vi "SC Save Modified VIs.vi"(8 "error in (no error)":errorcluster, 9 "project folder":path, 10 "project application":refnum<vi>) -> (0 "error out":errorcluster, 1 "cancelled?":bool)   [LabVIEW 2023]
doc: "Before a deploy: lists the VIs in the project's application instance (project application, from SC Get Project) that are inside the project folder and have unsaved changes, and the untitled (never saved) VIs there, asks Save All / Cancel, then asks where to save each untitled VI (starting in the project folder) and saves them all. Untitled VIs are saved first, because saving a caller of an untitled subVI fails. Cancelling any of it cancels the deploy. Unless cancelled, also saves the active project (LabVIEW has no public 'project modified' property)."
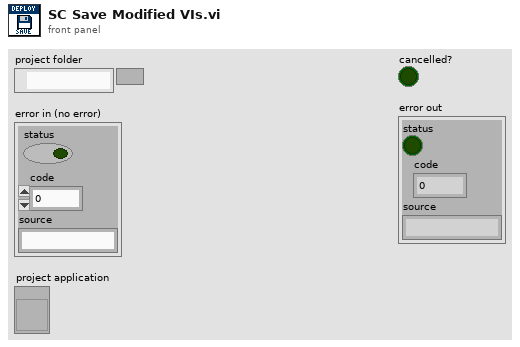
[diagram p1: front panel]
types:
  T1 = enum32{"existing file", "new file", "new or existing file", "existing dir", "new dir", "new or existing dir", "existing file (use LLBs)", "new file (use LLBs)", "new or existing file (use LLBs)", "new or existing file or directory (use LLBs)", "existing dir (use LLBs)", "new dir (use LLBs)", "new or existing dir (use LLBs)", "existing file or dir", "new file or dir", "new or existing file or dir", "existing file or dir (use LLBs)", "new file or dir (use LLBs)", "multi-select", "multi-select (use LLBs)"}
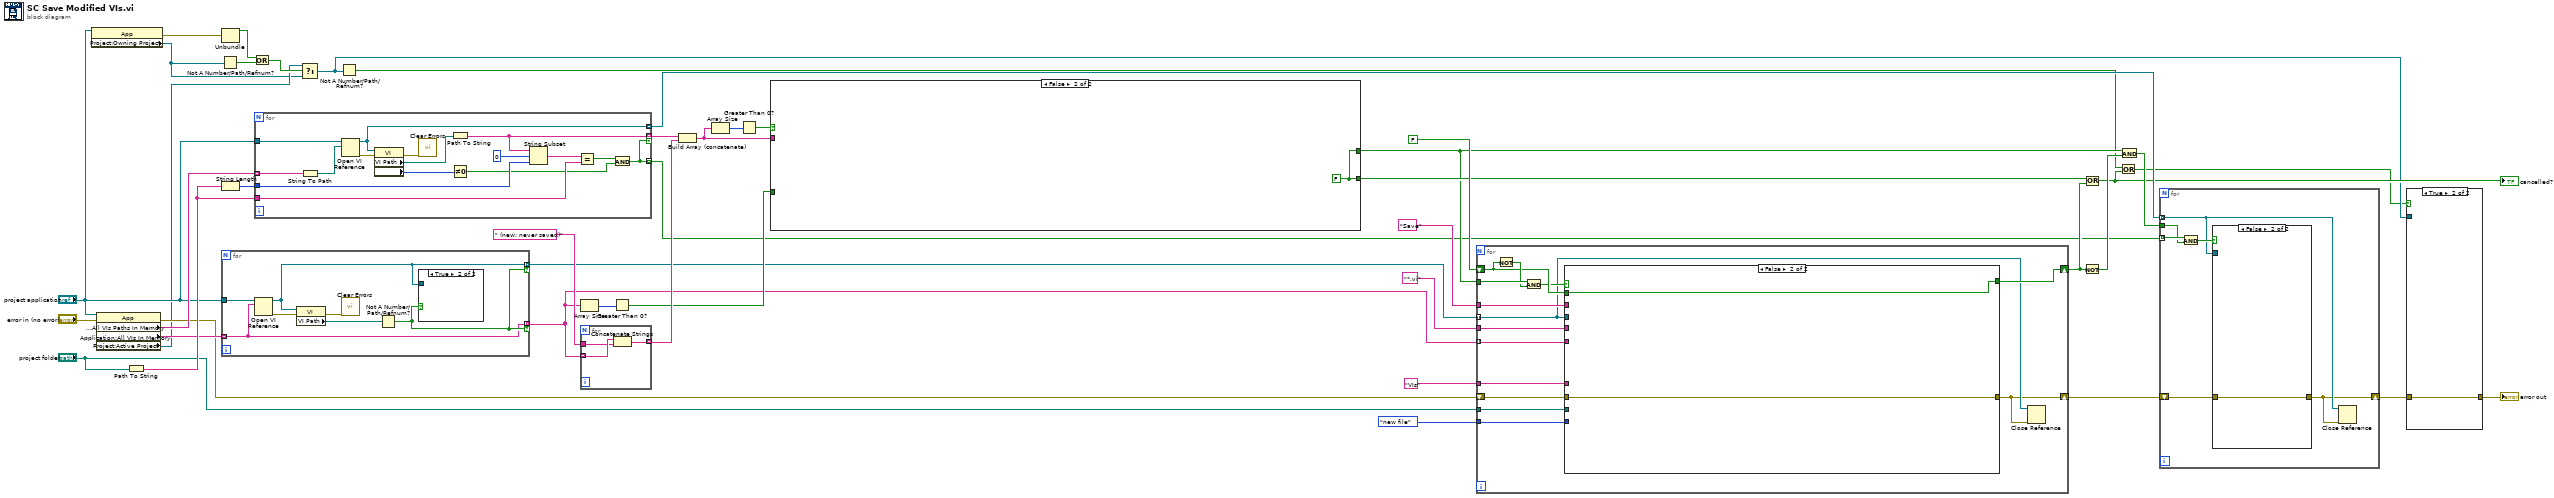
[diagram p0: block diagram]
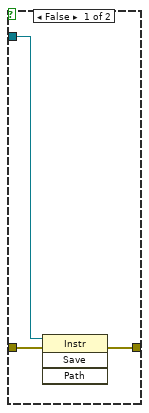
[diagram p2: hidden frame]
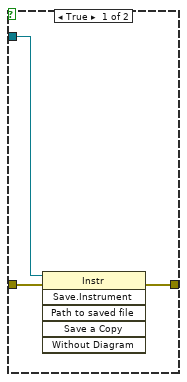
[diagram p3: hidden frame]
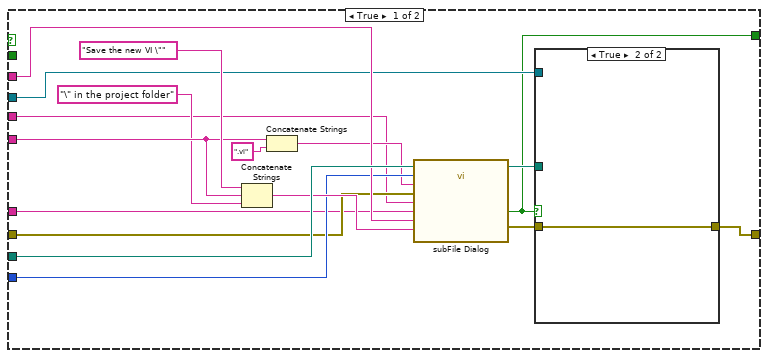
[diagram p4: hidden frame]
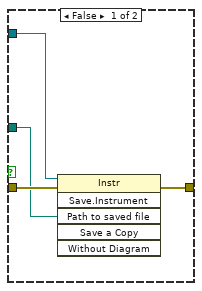
[diagram p5: hidden frame]
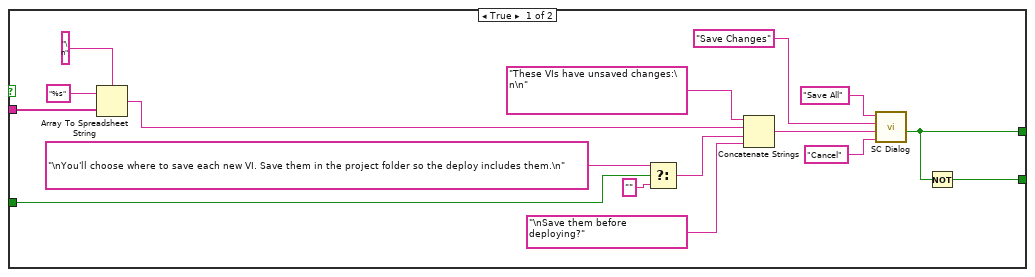
[diagram p6: hidden frame]
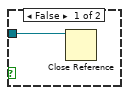
[diagram p7: hidden frame]
diagram:
  n1 = property class="App"(reference="project application") -> (error out=w12:errorcluster, "Project:Owning Project"=w7:refnum<vi>)  [unwired: 1 in, 1 out]
  n2 = property class="App"(reference="project application", error in="error in (no error)") -> (error out=w23:errorcluster, "Application:All VIs Paths In Memory"=w42:string[], "Application:All VIs In Memory"=w39:string[], "Project:Active Project"=w8:refnum<vi>)  [unwired: 1 out]
  n3 = Path To String(path="project folder") -> (string=w41:string)
  n4 = Not A Number/Path/Refnum?(number/path/refnum=w7) -> (NaN/Path/Refnum?=w10:bool)
  n5 = Unbundle(w12) -> ("status"=w11:bool)  [unwired: 2 out]
  n6 = String Length(string=w41) -> (length=w40:i32)
  n7 = for {
    tunnel: w39 -> [w44] mode=indexing
    tunnel: "project application" -> [w50]
    tunnel: [w46] -> w30 mode=indexing if=w45
    tunnel: [w44] -> w29 mode=indexing if=w45
    n8 = Open VI Reference(application reference (local)=w50, vi path=w44) -> (vi reference=w46:refnum<vi>, error out=w49:errorcluster)  [unwired: 4 in]
    n9 = property class="VI"(reference=w46, error in=w49) -> (error out=w48:errorcluster, "VI Path"=w47:path)  [unwired: 1 out]
    n10 = call <vilib>:"Clear Errors.vi"("error in (no error)"=w48) -> ()  [unwired: 5 in, 2 out]
    n11 = Not A Number/Path/Refnum?(number/path/refnum=w47) -> (NaN/Path/Refnum?=w45:bool)
    n12 = case shown="True" w45 {
      tunnel: w46 -> [w51 _]
      frame False {
        n13 = Close Reference(reference=w51) -> ()  [unwired: 1 in, 1 out]
      }
      frame True {
      }
    }
  }
  n14 = Or(x=w11, y=w10) -> (x .or. y?=w9:bool)
  n15 = for {
    tunnel: w42 -> [w67] mode=indexing
    tunnel: w41 -> [w58]
    tunnel: w40 -> [w60]
    tunnel: "project application" -> [w66]
    tunnel: [w54] -> w17 mode=indexing
    tunnel: [w53] -> w16 mode=indexing
    tunnel: [w52] -> w37 mode=indexing if=w53
    n16 = String To Path(string=w67) -> (path=w65:path)
    n17 = Open VI Reference(application reference (local)=w66, vi path=w65) -> (vi reference=w54:refnum<vi>, error out=w64:errorcluster)  [unwired: 4 in]
    n18 = property class="VI"(reference=w54, error in=w64) -> (error out=w63:errorcluster, "VI Path"=w62:path, "Modifications:VI Modifications Bitset"=w57:u64)  [unwired: 1 out]
    n19 = call <vilib>:"Clear Errors.vi"("error in (no error)"=w63) -> ()  [unwired: 5 in, 2 out]
    n20 = Path To String(path=w62) -> (string=w52:string)
    n21 = Not Equal To 0?(x=w57) -> (x != 0?=w55:bool)
    n22 = String Subset(string=w52, offset (0)=0, length (rest)=w60) -> (substring=w59:string)
    n23 = Equal?(x=w59, y=w58) -> (x = y?=w56:bool)
    n24 = And(x=w56, y=w55) -> (x .and. y?=w53:bool)
  }
  n25 = Select(t=w8, s=w9, f=w7) -> (s? t:f=w4:refnum<vi>)
  n26 = Not A Number/Path/Refnum?(number/path/refnum=w4) -> (NaN/Path/Refnum?=w6:bool)
  n27 = Array Size(array=w29) -> (size(s)=w35:i32)
  n28 = for {
    tunnel: w29 -> [w70] mode=indexing
    tunnel: " (new: never saved)" -> [w69]
    tunnel: [w68] -> w36 mode=indexing
    n29 = Concatenate Strings(w70, w69) -> (w68:string)
  }
  n30 = Greater Than 0?(x=w35) -> (x > 0?=w32:bool)
  n31 = Build Array (concatenate)(w37, w36) -> (w33:string[])
  n32 = Array Size(array=w33) -> (size(s)=w34:i32)
  n33 = Greater Than 0?(x=w34) -> (x > 0?=w31:bool)
  n34 = case shown="False" w31 {
    tunnel: w33 -> [w85 _]
    tunnel: w32 -> [w83 _]
    tunnel: [w72 w87] -> w19
    tunnel: [w71 w87] -> w21
    frame True {
      n35 = Array To Spreadsheet String(delimiter (Tab)="\n", array=w85, 3:"%s") -> (spreadsheet string=w79:string)
      n36 = Select(t="\nYou'll choose where to save each new VI. Save them in the project folder so the deploy includes them.\n", s=w83, f="") -> (s? t:f=w78:string)
      n37 = Concatenate Strings("These VIs have unsaved changes:\n\n", w79, w78, "\nSave them before deploying?") -> (w76:string)
      n38 = call "SC Dialog.vi"("Cancel text"="Cancel", "message"=w76, "window title"="Save Changes", "OK text"="Save All") -> ("OK?"=w72:bool)  [unwired: 7 in]
      n39 = Not(x=w72) -> (.not. x?=w71:bool)
    }
    frame False {
      w87 = FALSE
    }
  }
  n40 = for {
    tunnel: w30 -> [w89] mode=indexing
    tunnel: w29 -> [w99] mode=indexing
    tunnel: w19 -> [w101]
    tunnel: "project folder" -> [w98]
    tunnel: "*.vi" -> [w95]
    tunnel: "VIs" -> [w94]
    tunnel: "Save" -> [w93]
    tunnel: T1."new file" -> [w92]
    shift-right: [w88] -> w14
    shift-left: w23 -> [w97]
    shift-right: [w91] -> w20
    shift-left: FALSE -> [w96]
    n41 = Not(x=w96) -> (.not. x?=w100:bool)
    n42 = And(x=w101, y=w100) -> (x .and. y?=w90:bool)
    n43 = case shown="False" w90 {
      tunnel: w89 -> [w106 _]
      tunnel: w99 -> [w116 _]
      tunnel: w98 -> [w114 _]
      tunnel: w97 -> [w109 w125]
      tunnel: w96 -> [_ w124]
      tunnel: w95 -> [w108 _]
      tunnel: w94 -> [w107 _]
      tunnel: w93 -> [w112 _]
      tunnel: w92 -> [w111 _]
      tunnel: [w103 w125] -> w88
      tunnel: [w102 w124] -> w91
      frame True {
        n44 = Concatenate Strings("Save the new VI \"", w116, "\" in the project folder") -> (w113:string)
        n45 = Concatenate Strings(w116, ".vi") -> (w110:string)
        n46 = call <vilib>:"subFile Dialog.vi"("start path"=w114, "prompt"=w113, "button label"=w112, "selection mode"=w111, "default name"=w110, "error in"=w109, "pattern (all files)"=w108, "pattern label"=w107) -> ("selected path"=w105:path, "cancelled"=w102:bool, "error out"=w104:errorcluster)  [unwired: 3 in, 2 out]
        n47 = case shown="True" w102 {
          tunnel: w106 -> [w122 _]
          tunnel: w105 -> [w120 _]
          tunnel: w104 -> [w121 w123]
          tunnel: [w119 w123] -> w103
          frame False {
            n48 = invoke class="Instr" method="Save.Instrument"(reference=w122, error in=w121, "Path to saved file"=w120) -> (error out=w119:errorcluster)  [unwired: 3 in, 5 out]
          }
          frame True {
          }
        }
      }
      frame False {
      }
    }
    n49 = Close Reference(reference=w89, error in (no error)=w88) -> ()  [unwired: 1 out]
  }
  n50 = Or(x=w21, y=w20) -> (x .or. y?=w5:bool)
  "cancelled?" <- w5
  n51 = Not(x=w20) -> (.not. x?=w18:bool)
  n52 = Or(x=w6, y=w5) -> (x .or. y?=w1:bool)
  n53 = And(x=w19, y=w18) -> (x .and. y?=w15:bool)
  n54 = for {
    tunnel: w17 -> [w127] mode=indexing
    tunnel: w16 -> [w131] mode=indexing
    tunnel: w15 -> [w130]
    shift-right: [w126] -> w3
    shift-left: w14 -> [w129]
    n55 = And(x=w131, y=w130) -> (x .and. y?=w128:bool)
    n56 = case shown="False" w128 {
      tunnel: w127 -> [w134 _]
      tunnel: w129 -> [w133 w135]
      tunnel: [w132 w135] -> w126
      frame True {
        n57 = invoke class="Instr" method="Save.Instrument"(reference=w134, error in=w133) -> (error out=w132:errorcluster)  [unwired: 4 in, 5 out]
      }
      frame False {
      }
    }
    n58 = Close Reference(reference=w127, error in (no error)=w126) -> ()  [unwired: 1 out]
  }
  n59 = case shown="True" w1 {
    tunnel: w4 -> [w138 _]
    tunnel: w3 -> [w137 w139]
    tunnel: [w136 w139] -> w2
    frame False {
      n60 = invoke class="Instr" method="Save"(reference=w138, error in=w137) -> (error out=w136:errorcluster)  [unwired: 2 in, 3 out]
    }
    frame True {
    }
  }
  "error out" <- w2
